vi "MQTT String - Validate UTF-8.vi"(11 "UTF-8 Data":u8[](array[numeric])) -> (2 "Valid":bool)   [LabVIEW 2019, in "KoRE-MQTT.lvlib"]
doc: "Copyright (c) 2025 KoRElibs.com\nSPDX-License-Identifier: EUPL-1.2\n\nThis VI is licensed under the European Union Public License (EUPL) Version 1.2. You may use this VI unmodified in proprietary works. If you distribute a modified version of this file, the modified file must be released under the EUPL-1.2. Full license: https://joinup.ec.europa.eu/asset/eupl/eupl/1.2/"
uses:
  KoRE-MQTT.lvlib
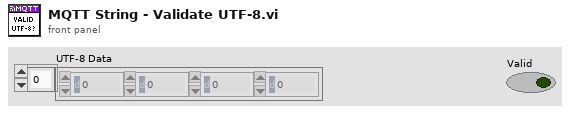
[diagram p1: front panel]
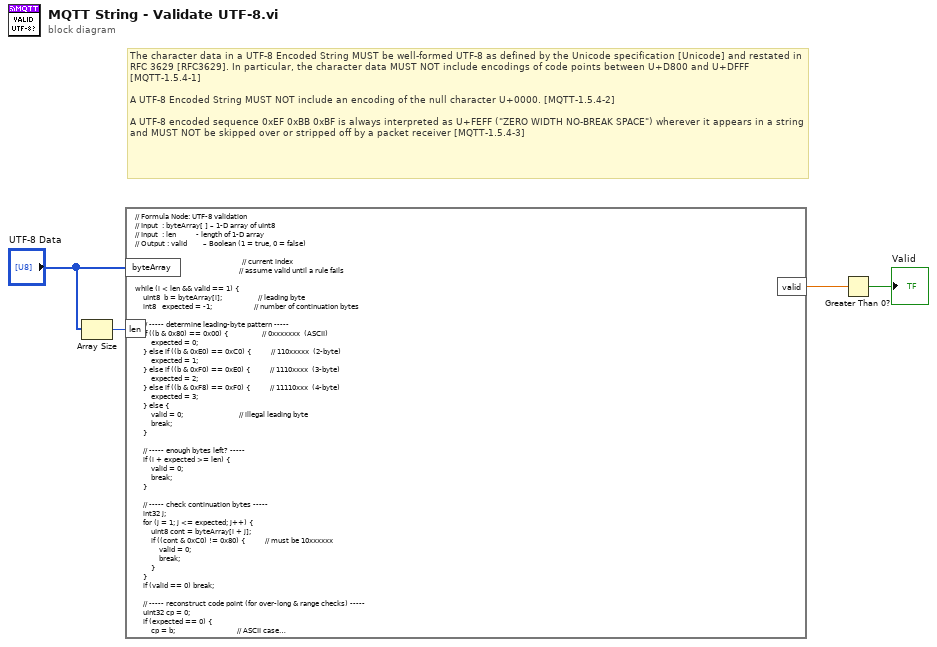
[diagram p0: block diagram]
diagram:
  # "The character data in a UTF-8 Encoded String MUST be well-formed UTF-8 as defined by the Unicode specification [Unicode] and restated in RFC 3629 [RFC3629]. In particular, the character data MUST NOT include encodings of code points between U+D800 and U+DFFF [MQTT-1.5.4-1]\n\nA UTF-8 Encoded String MUST NOT include an encoding of the null character U+0000. [MQTT-1.5.4-2]\n\nA UTF-8 encoded sequence 0xEF 0xBB 0xBF is always interpreted as U+FEFF (\"ZERO WIDTH NO-BREAK SPACE\") wherever it appears in a string and MUST NOT be skipped over or stripped off by a packet receiver [MQTT-1.5.4-3]"
  n1 = Array Size(array="UTF-8 Data") -> (size(s)=w1:i32)
  n2 = formula code="// Formula Node: UTF-8 validation\n// Input  : byteArray[ ] – 1-D array of uInt8\n// Input  : len          - length of 1-D array\n// Output : valid        – Boolean (1 = true, 0 = false)\n\nuInt32 i = 0;                                 // current index\nvalid = 1;                                    // assume valid until a rule fails\n\nwhile (i < len && valid == 1) {\n    uInt8  b = byteArray[i];                  // leading byte\n    int8   expected = -1;                     // number of continuation bytes\n\n    // ----- determine leading-byte pattern -----\n    if ((b & 0x80) == 0x00) {                 // 0xxxxxxx  (ASCII)\n        expected = 0;\n    } else if ((b & 0xE0) == 0xC0) {          // 110xxxxx  (2-byte)\n        expected = 1;\n    } else if ((b & 0xF0) == 0xE0) {          // 1110xxxx  (3-byte)\n        expected = 2;\n    } else if ((b & 0xF8) == 0xF0) {          // 11110xxx  (4-byte)\n        expected = 3;\n    } else {\n        valid = 0;                            // illegal leading byte\n        break;\n    }\n\n    // ----- enough bytes left? -----\n    if (i + expected >= len) {\n        valid = 0;\n        break;\n    }\n\n    // ----- check continuation bytes -----\n    int32 j;\n    for (j = 1; j <= expected; j++) {\n        uInt8 cont = byteArray[i + j];\n        if ((cont & 0xC0) != 0x80) {          // must be 10xxxxxx\n            valid = 0;\n            break;\n        }\n    }\n    if (valid == 0) break;\n\n    // ----- reconstruct code point (for over-long & range checks) -----\n    uInt32 cp = 0;\n    if (expected == 0) {\n        cp = b;                               // ASCII case\n    } else {\n        // mask off the leading bits of the first byte\n        uInt8 mask = 0xFF >> (expected + 2);\n        cp = b & mask;\n        for (j = 1; j <= expected; j++) {\n            cp = (cp << 6) | (byteArray[i + j] & 0x3F);\n        }\n    }\n\n    // ----- reject over-long encodings -----\n    if ( (cp <= 0x7F && expected > 0) ||\n         (cp <= 0x7FF && expected > 1) ||\n         (cp <= 0xFFFF && expected > 2) ) {\n        valid = 0;\n        break;\n    }\n\n    // ----- reject illegal Unicode ranges -----\n    if (cp > 0x10FFFF || (cp >= 0xD800 && cp <= 0xDFFF)) {\n        valid = 0;\n        break;\n    }\n\n    // ----- advance to next character -----\n    i = i + expected + 1;\n}\n\n// End while – valid stays 1 only if every byte passed all tests"("byteArray"="UTF-8 Data", "len"=w1) -> ("valid"=w4:dbl)
  n3 = Greater Than 0?(x=w4) -> (x > 0?=→"Valid":bool)
